vi "Sync.vi"(8 "error in (no error)":errorcluster, 10 "file ref":refnum<file>, 11 "rollover trigger in":refnum<class "RolloverTrigger.Multi.lvclass">) -> (0 "error out":errorcluster, 3 "rollover trigger out":refnum<class "RolloverTrigger.Multi.lvclass">)   [LabVIEW 2018, in "GLog.lvlib" / "RolloverTrigger.Multi.lvclass"]
doc: "Synchronizes the rollover trigger with the new file."
uses:
  RolloverTrigger.Multi.lvclass
  RolloverTrigger.Multi.lvclass/RolloverTrigger.Multi.ctl
  RolloverTrigger/RolloverTrigger.lvclass
panel:
  # "Connector Pane"
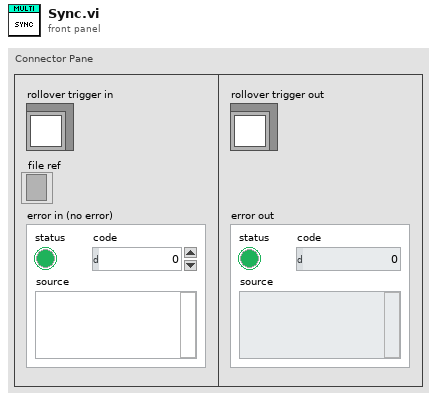
[diagram p1: front panel]
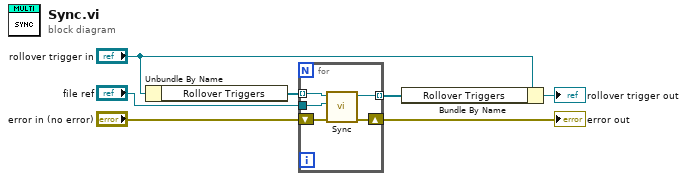
[diagram p0: block diagram]
diagram:
  n1 = Unbundle By Name("rollover trigger in") -> ("Rollover Triggers"=w7:refnum<class "RolloverTrigger.lvclass">[])
  n2 = for {
    tunnel: w7 -> [w12] mode=indexing
    tunnel: [w11] -> w6 mode=indexing
    shift-right: [w9] -> w2
    shift-left: "error in (no error)" -> [w10]
    tunnel: "file ref" -> [w8]
    n3 = call-dynamic "Sync.vi"("error in (no error)"=w10, "file ref"=w8, "rollover trigger in"=w12) -> ("error out"=w9:errorcluster, "rollover trigger out"=w11:refnum<class "RolloverTrigger.lvclass">)  [unwired: 7 in]
  }
  "error out" <- w2
  n4 = Bundle By Name(cluster="rollover trigger in", "Rollover Triggers"=w6) -> (→"rollover trigger out":refnum<class "RolloverTrigger.Multi.lvclass">)
